vi "Pat message.vi"(8 "error in (no error)":errorcluster, 11 "Guardian in":refnum<class "Guardian.lvclass">) -> (0 "error out":errorcluster, 1 "Data":string[](array[string]), 2 "Message name":string, 3 "Guardian out":refnum<class "Guardian.lvclass">)   [LabVIEW 2020, in "TALOS.lvlib" / "Guardian.lvlib" / "Guardian.lvclass"]
uses:
  Guardian.lvclass
  C:/LabVIEW Code/TALOS/talos/Ancestor/Ancestor/Ancestor.lvclass
  Ancestor/Ancestor/Ancestor.lvclass/Ancestor.ctl
  Guardian.lvclass/Guardian.ctl
  Ancestor/Ancestor/Ancestor.lvclass
  TALOS.lvlib
  C:/LabVIEW Code/TALOS/builds/Actor Framework PPL/Actor Framework.lvlibp/1abvi3w/vi.lib/ActorFramework/Actor/Actor.lvclass
  C:/LabVIEW Code/TALOS/talos/Guardian/Guardian/Guardian.lvclass
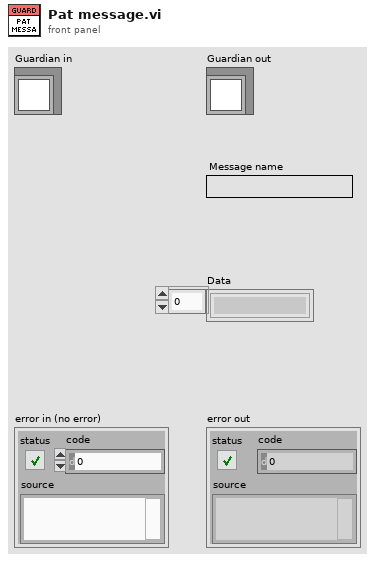
[diagram p1: front panel]
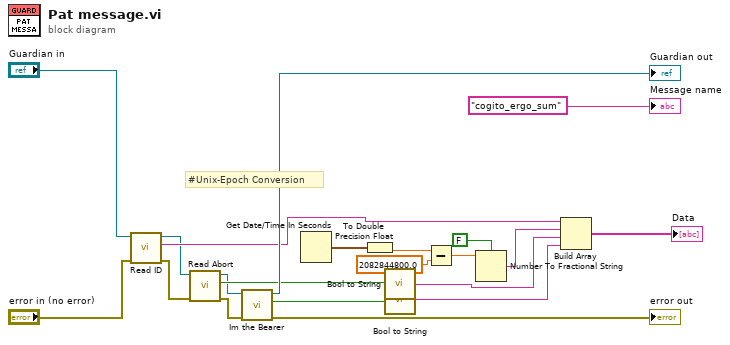
[diagram p0: block diagram]
diagram:
  # "#Unix-Epoch Conversion"
  n1 = call "Read ID.vi"("error in (no error)"="error in (no error)", "Ancestor in"="Guardian in") -> ("error out"=w12:errorcluster, "ID"=w19:string, "Ancestor out"=w13:refnum<class "Guardian.lvclass">)  [unwired: 7 in]
  n2 = call "Read Abort.vi"("error in (no error)"=w12, "Guardian in"=w13) -> ("error out"=w11:errorcluster, "Abort"=w14:bool, "Guardian out"=w10:refnum<class "Guardian.lvclass">)  [unwired: 7 in]
  n3 = call "Im the Bearer.vi"("error in (no error)"=w11, "Guardian in"=w10) -> ("error out"=→"error out":errorcluster, "I'm the Bearer"=w15:bool, "Guardian out"=→"Guardian out":refnum<class "Guardian.lvclass">)  [unwired: 7 in]
  n4 = Get Date/Time In Seconds() -> (seconds since 1Jan1904=w20:timestamp)
  n5 = To Double Precision Float(number=w20) -> (double precision float=w7:dbl)
  n6 = call "Bool to String.vi"("Boolean"=w14) -> ("String"=w3:string)
  n7 = call "Bool to String.vi"("Boolean"=w15) -> ("String"=w2:string)
  n8 = Subtract(x=w7, y=2082844800.0) -> (x-y=w6:dbl)
  n9 = Number To Fractional String(use system decimal point (T)=FALSE, number=w6) -> (F-format string=w4:string)  [unwired: 2 in]
  n10 = Build Array(w19, w4, w3, w2) -> (→"Data":string[])
  "Message name" <- "cogito_ergo_sum" ("Message")
